vi "ini_Read_Write.vi"(0 "?":T1, 5 "Write Section":string, 7 "Write key":string="Access", 9 "Write":string, 11 "error in (no error) 2":errorcluster, 12 "Read Section":string, 13 "Read Key":string="A") -> (4 "value":string, 15 "error in (no error) 3":errorcluster)   [LabVIEW 2021]
uses:
  Control/Ini.ctl
  <vilib>/Utility/config.llb/Write Key (String).vi
  <vilib>/Utility/config.llb/Read Key (String).vi
  <vilib>/Utility/config.llb/NI_LVConfig.lvlib
panel:
  out "appended path":path
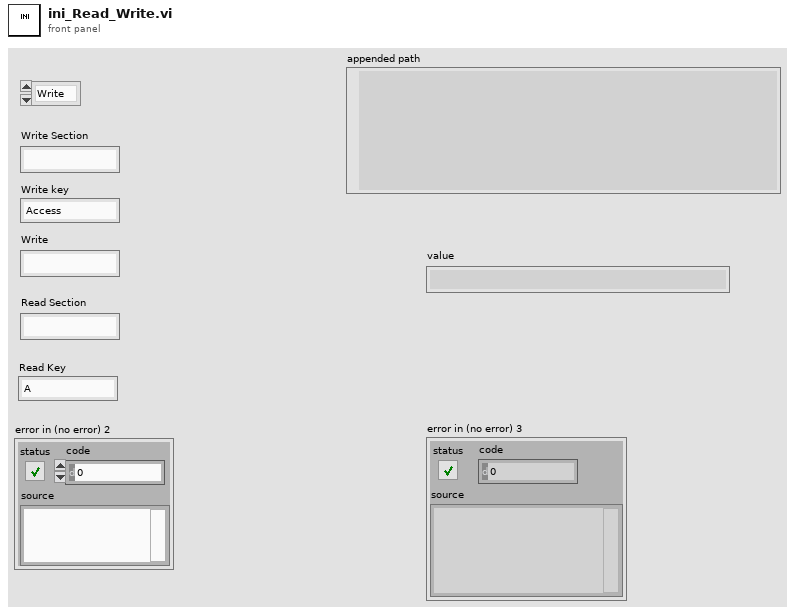
[diagram p1: front panel]
types:
  T1 = typedef "Ini.ctl" = enum16{"Write", "Read"}
  T2 = typedef "NI_LVConfig.lvlib/Config Data RefNum.ctl" = refnum<k1>
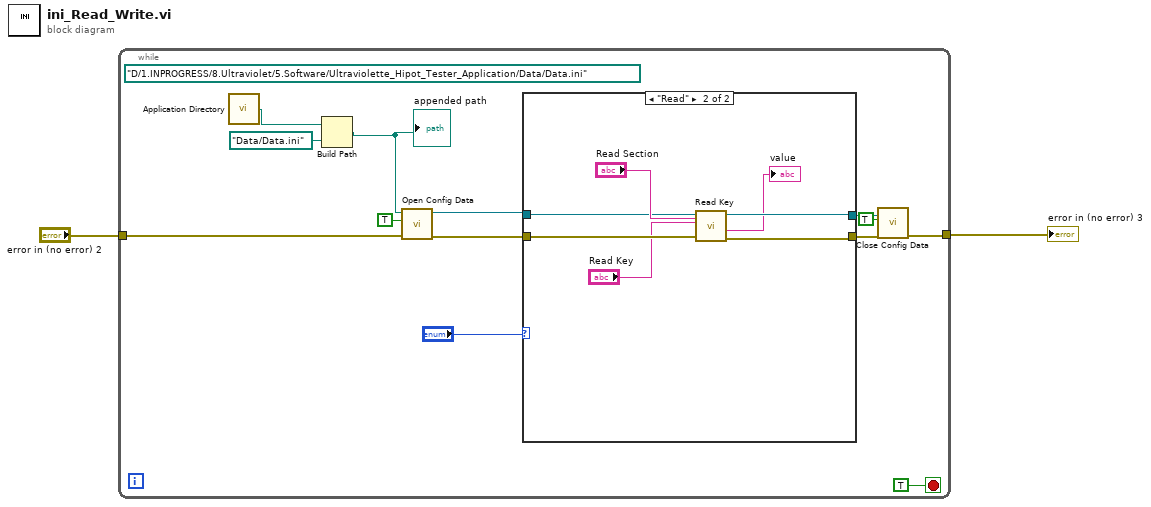
[diagram p0: block diagram]
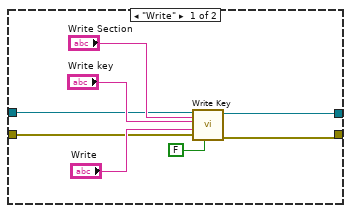
[diagram p2: hidden frame]
diagram:
  n1 = while {
    tunnel: [w8] -> w1
    tunnel: "error in (no error) 2" -> [w11]
    stop <- TRUE stop-if-true
    (unwired) path "D:/1.INPROGRESS/8.Ultraviolet/5.Software/Ultraviolette_Hipot_Tester_Application/Data/Data.ini" ("base path")
    n2 = call <vilib>:"Application Directory.vi"() -> ("Application Directory"=w4:path)
    n3 = Build Path(base path=w4, name or relative path=path "Data/Data.ini") -> (appended path=w3:path)
    "appended path" <- w3
    n4 = call <vilib>:"Open Config Data.vi"("error in (no error)"=w11, "create file if necessary (T)"=TRUE, "configuration file path"=w3) -> ("error out"=w10:errorcluster, "refnum"=w12:T2)  [unwired: 6 in, 1 out]
    n5 = case shown="\"Read\"" "?" {
      tunnel: [w20 w30] -> w13
      tunnel: w12 -> [w19 w27]
      tunnel: w10 -> [w18 w26]
      tunnel: [w17 w25] -> w9
      frame "Write" {
        n6 = call-poly <vilib>:"Write Key.vi"("write raw string? (F)"=FALSE, "section"="Write Section", "error in (no error)"=w18, "value"="Write", "key"="Write key", "refnum"=w19) -> ("error out"=w17:errorcluster, "refnum out"=w20:T2)  [unwired: 3 in, 1 out]
      }
      frame "Read" {
        n7 = call-poly <vilib>:"Read Key.vi"("section"="Read Section", "error in (no error)"=w26, "key"="Read Key", "refnum"=w27) -> ("error out"=w25:errorcluster, "value"=→"value":string, "refnum out"=w30:T2)  [unwired: 4 in, 1 out]
      }
    }
    n8 = call <vilib>:"Close Config Data.vi"("error in (no error)"=w9, "write file if changed (T)"=TRUE, "refnum"=w13) -> ("error out"=w8:errorcluster)  [unwired: 7 in, 1 out]
  }
  "error in (no error) 3" <- w1
